vi "TXT to TDMS Q.vi"(8 "error in":errorcluster caption="エラー入力（エラーなし）", 9 "数値":dbl=-1.0 format="%#_13g", 11 "Original File name (TXT)":path) -> (0 "error out":errorcluster caption="エラー出力", 3 "Raw data Graph":dbl[](graph))   [LabVIEW 2018]
uses:
  <vilib>/Utility/file.llb/Read Delimited Spreadsheet (DBL).vi
panel:
  out "x = y?":bool
  out "lowercase file extension":string caption="小文字ファイル拡張子"
  out "first row":dbl[](array[numeric]) caption="最初の行"
  out "file or folder exists?":bool caption="既存するファイルまたはフォルダ?"
  out "Create File name (TDMS)":path
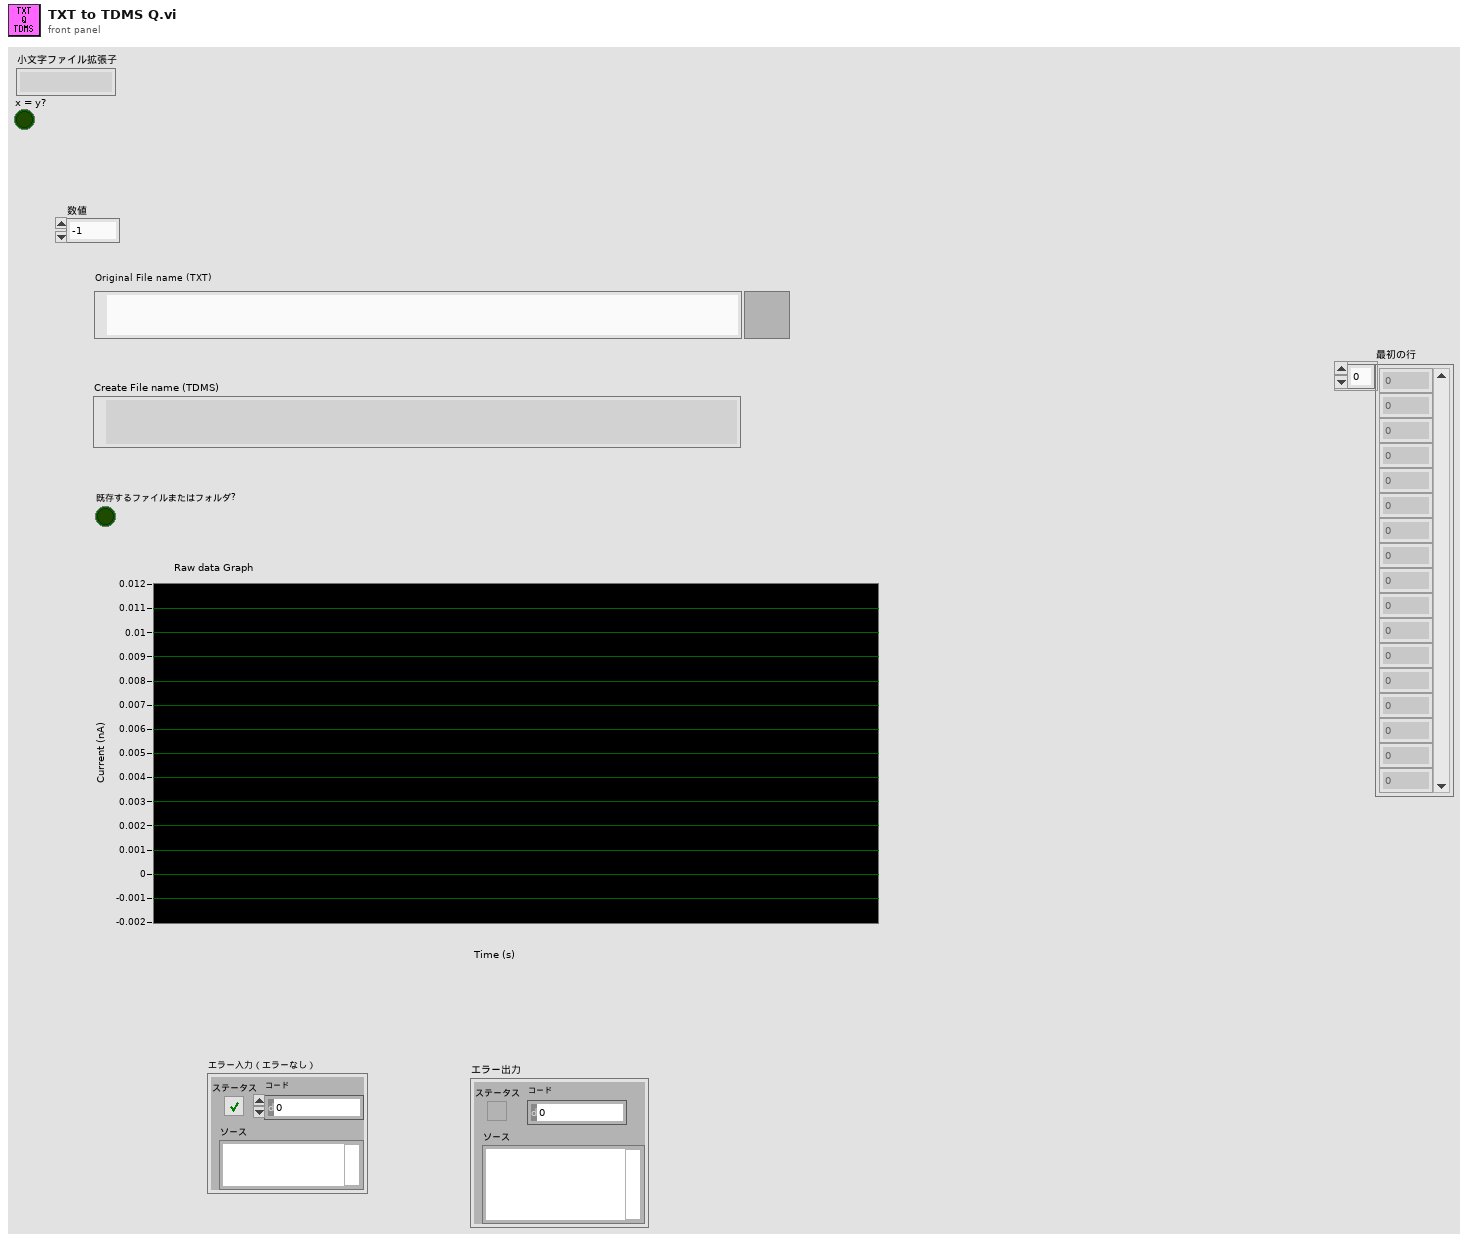
[diagram p1: front panel]
types:
  T1 = enum16{"open", "open or create", "create or replace", "create", "open (read-only)"}
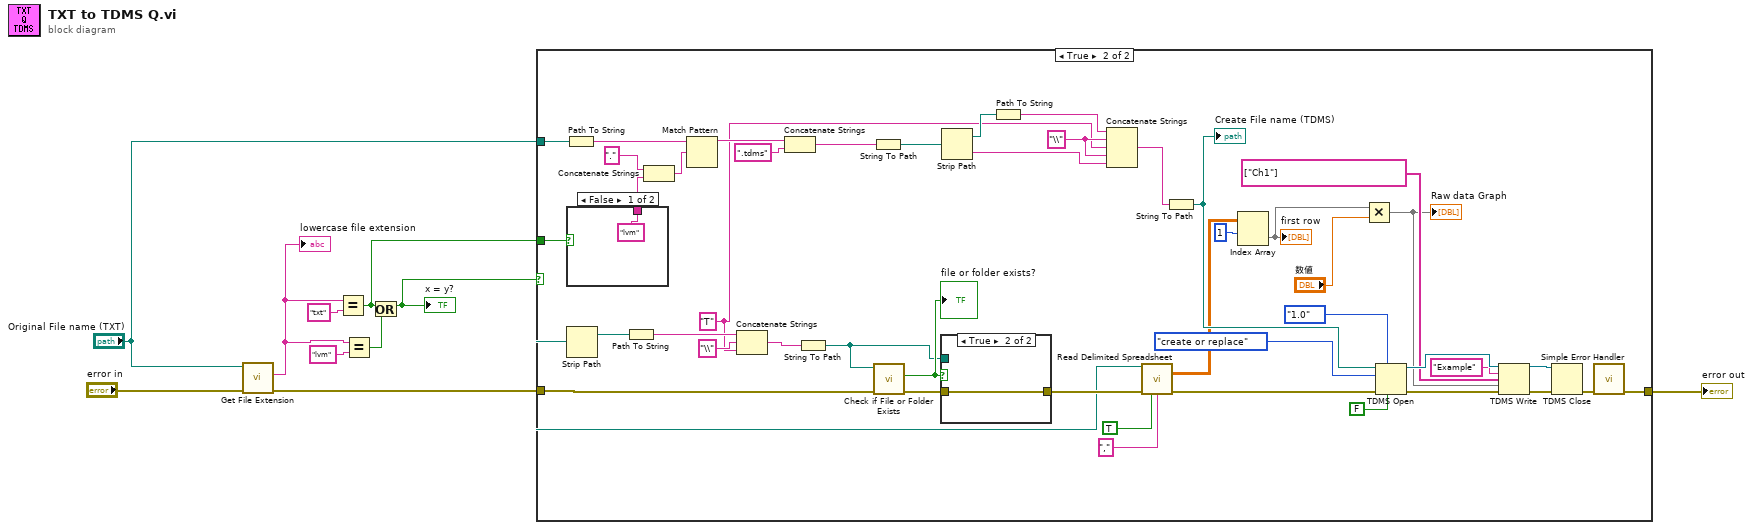
[diagram p0: block diagram]
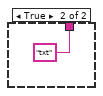
[diagram p3: hidden frame]
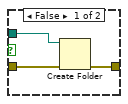
[diagram p4: hidden frame]
diagram:
  n1 = call <vilib>:"Get File Extension.vi"("error in (no error)"="error in", "file"="Original File name (TXT)") -> ("error out"=w6:errorcluster, "lowercase file extension"=w4:string)  [unwired: 5 in, 3 out]
  "lowercase file extension" <- w4
  n2 = Equal?(x=w4, y="txt") -> (x = y?=w1:bool)
  n3 = Equal?(x=w4, y="lvm") -> (x = y?=w2:bool)
  n4 = Or(x=w1, y=w2) -> (x .or. y?=w3:bool)
  "x = y?" <- w3
  n5 = case shown="True" w3 {
    tunnel: [w11 w31] -> w10
    tunnel: "Original File name (TXT)" -> [_ w14]
    tunnel: w6 -> [w11 w13]
    tunnel: w1 -> [_ w12]
    frame False {
    }
    frame True {
      w21 = "T" ("Folder Name")
      w44 = "\\" ("文字列")
      n6 = Path To String(path=w14) -> (string=w56:string)
      n7 = case shown="False" w12 {
        tunnel: ["lvm" ("File Extention form") "txt" ("File Extention form")] -> w52
        frame False {
        }
        frame True {
        }
      }
      n8 = Strip Path(path=w14) -> (stripped path=w24:path)  [unwired: 1 out]
      n9 = Path To String(path=w24) -> (string=w23:string)
      n10 = Concatenate Strings("." ("正規表現"), w52) -> (w51:string)
      n11 = Match Pattern(string=w56, regular expression=w51) -> (before substring=w55:string)  [unwired: 1 in, 3 out]
      n12 = Concatenate Strings(w23, "\\" ("文字列"), w21) -> (w27:string)
      n13 = Concatenate Strings(w55, ".tdms" ("文字列")) -> (w54:string)
      n14 = String To Path(string=w27) -> (path=w28:path)
      n15 = String To Path(string=w54) -> (path=w50:path)
      n16 = call <vilib>:"Check if File or Folder Exists.vi"("error in (no error)"=w13, "path"=w28) -> ("error out"=w26:errorcluster, "file or folder exists?"=w29:bool)  [unwired: 7 in, 1 out]
      "file or folder exists?" <- w29
      n17 = case shown="True" w29 {
        tunnel: w28 -> [w61 _]
        tunnel: w26 -> [w60 w62]
        tunnel: [w59 w62] -> w25
        frame False {
          n18 = Create Folder(path (use dialog)=w61, error in=w60) -> (error out=w59:errorcluster)  [unwired: 1 in, 2 out]
        }
        frame True {
        }
      }
      n19 = Strip Path(path=w50) -> (stripped path=w49:path, name=w45:string)
      n20 = Path To String(path=w49) -> (string=w48:string)
      n21 = Concatenate Strings(w48, w44, w21, w44, w45) -> (w47:string)
      n22 = call-poly <vilib>:"Read Delimited Spreadsheet.vi"("file path (dialog if empty)"=w14, "error in (no error)"=w25, "transpose? (F)"=TRUE ("transpose (no:F)"), "delimiter (\\t)"="," ("delimiter (\\t)")) -> ("all rows"=w19:dbl[][], "error out"=w32:errorcluster)  [unwired: 6 in, 4 out]
      n23 = String To Path(string=w47) -> (path=w34:path)
      "Create File name (TDMS)" <- w34
      n24 = Index Array(array=w19, index (row)=1 ("指標 （行）")) -> (element=w17:dbl[])  [unwired: 1 in]
      "first row" <- w17
      n25 = Multiply(x=w17, y="数値") -> (x*y=w16:dbl[])
      "Raw data Graph" <- w16
      n26 = TDMS Open(6:FALSE ("disable buffering (T)"), 7:enum16{"1.0", "2.0"}."1.0" ("file format version (2.0)"), 8:w32, 10:T1."create or replace" ("operation"), 11:w34) -> (0:w39:errorcluster, 3:w40:refnum<k34>)  [unwired: 2 in]
      n27 = TDMS Write(0:w40, 5:"Example" ("group name in (Untitled)"), 7:string[] ["Ch1"] ("チャンネル名入力（名称未設定）"), 9:w16, 11:w39) -> (4:w43:refnum<k34>, 15:w42:errorcluster)  [unwired: 1 in, 2 out]
      n28 = TDMS Close(8:w42, 11:w43) -> (0:w35:errorcluster)  [unwired: 1 out]
      n29 = call <vilib>:"Simple Error Handler.vi"("error in (no error)"=w35) -> ("error out"=w31:errorcluster)  [unwired: 1 in, 7 out]
    }
  }
  "error out" <- w10
